vi "Drive Teleop Handler.vi"(10 "Call Context":T1=enum."Stop") -> ()   [LabVIEW 2027]
uses:
  Drive/Implementation/Driving Mode.ctl
  <vilib>/Rock Robotics/WPI/Joystick/XBox Buttons Indexer.ctl
  swerve-template/Type Definitions/Data/Robot Velocities.ctl
  fdc21bd4-9215-41b8-8367-bf19dde4ba27.vi
  <vilib>/Rock Robotics/Network Tables/NT Read Number.vi
  Framework/Robot Global Data.vi
  <vilib>/Rock Robotics/WPI/DriverStation/WPI_DriverStationDerivedRobotMode.ctl
  20f039dc-a6f5-4e97-88ba-31848a91c715.vi
  ce51abe2-3967-49ec-91df-d4b8ef358bb3.vi
  <vilib>/Rock Robotics/Network Tables/NT Read Boolean.vi
  2558f998-dd4e-4154-8f44-6f70b21d0474.vi
  <vilib>/Rock Robotics/Network Tables/NT Write Boolean.vi
  <vilib>/MRC/MrcLib.lvlib
panel:
  in  "Max ToF Data":cluster{"ToF":dbl, "Dist":dbl}={"ToF"=1.2, "Dist"=10.52}
  in  "Min ToF Data":cluster{"ToF":dbl, "Dist":dbl}={"ToF"=1.0, "Dist"=6.0}
  in  "Time in Flight":dbl=1.1
  in  "Max Translation Align":dbl=4.0
  in  "Deadband Info":T2={"Deadband"=0.05, "Deadband High"=1.0, "Deadband Low"=0.05}
  in  "Max Velocities":T3={"X Velocity"=15.0, "Y Velocity"=15.0, "Rotational \nVelocity"=270.0}
  in  "Sinusoidal Terms":cluster{"Max Velocity":dbl, "Frequency":dbl}
  in  "Teleop Mode":T4(ring)
  in  "Joystick Inputs":T5(array[cluster])
  in  "Send Inputs":bool
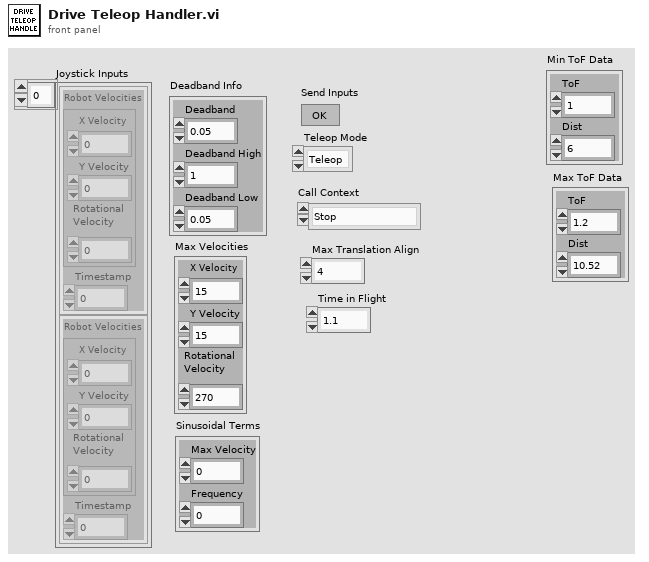
[diagram p1: front panel]
types:
  T1 = typedef "WPI_DriverStationDerivedRobotMode.ctl" = enum16{"Init", "Execute", "Stop"}
  T2 = cluster{"Deadband":dbl, "Deadband High":dbl, "Deadband Low":dbl}
  T3 = typedef "Robot Velocities.ctl" = cluster{"X Velocity":dbl, "Y Velocity":dbl, "Rotational \nVelocity":dbl}
  T4 = enum16{"Teleop", "Simulated Teleop", "Sine Velocity Profiles", "Circle Simulator"}
  T5 = cluster{"Robot Velocities":T3, "Timestamp":dbl}[]
  T6 = typedef "XBox Buttons Indexer.ctl" = enum16{"A", "B", "X", "Y", "Left Bumper", "Right Bumper", "Back", "Start", "Left Joystick", "Right Joystick"}
  T7 = typedef "Driving Mode.ctl" = enum16{"Robot Centric", "Field Centric"}
  T8 = typedef "WPI_JoystickDevRef.ctl" = cluster{"Device":T9}
  T9 = typedef "WPI_JoystickDeviceEnum.ctl" = enum16{"USB 0", "USB 1", "USB 2", "USB 3", "USB 4", "USB 5"}
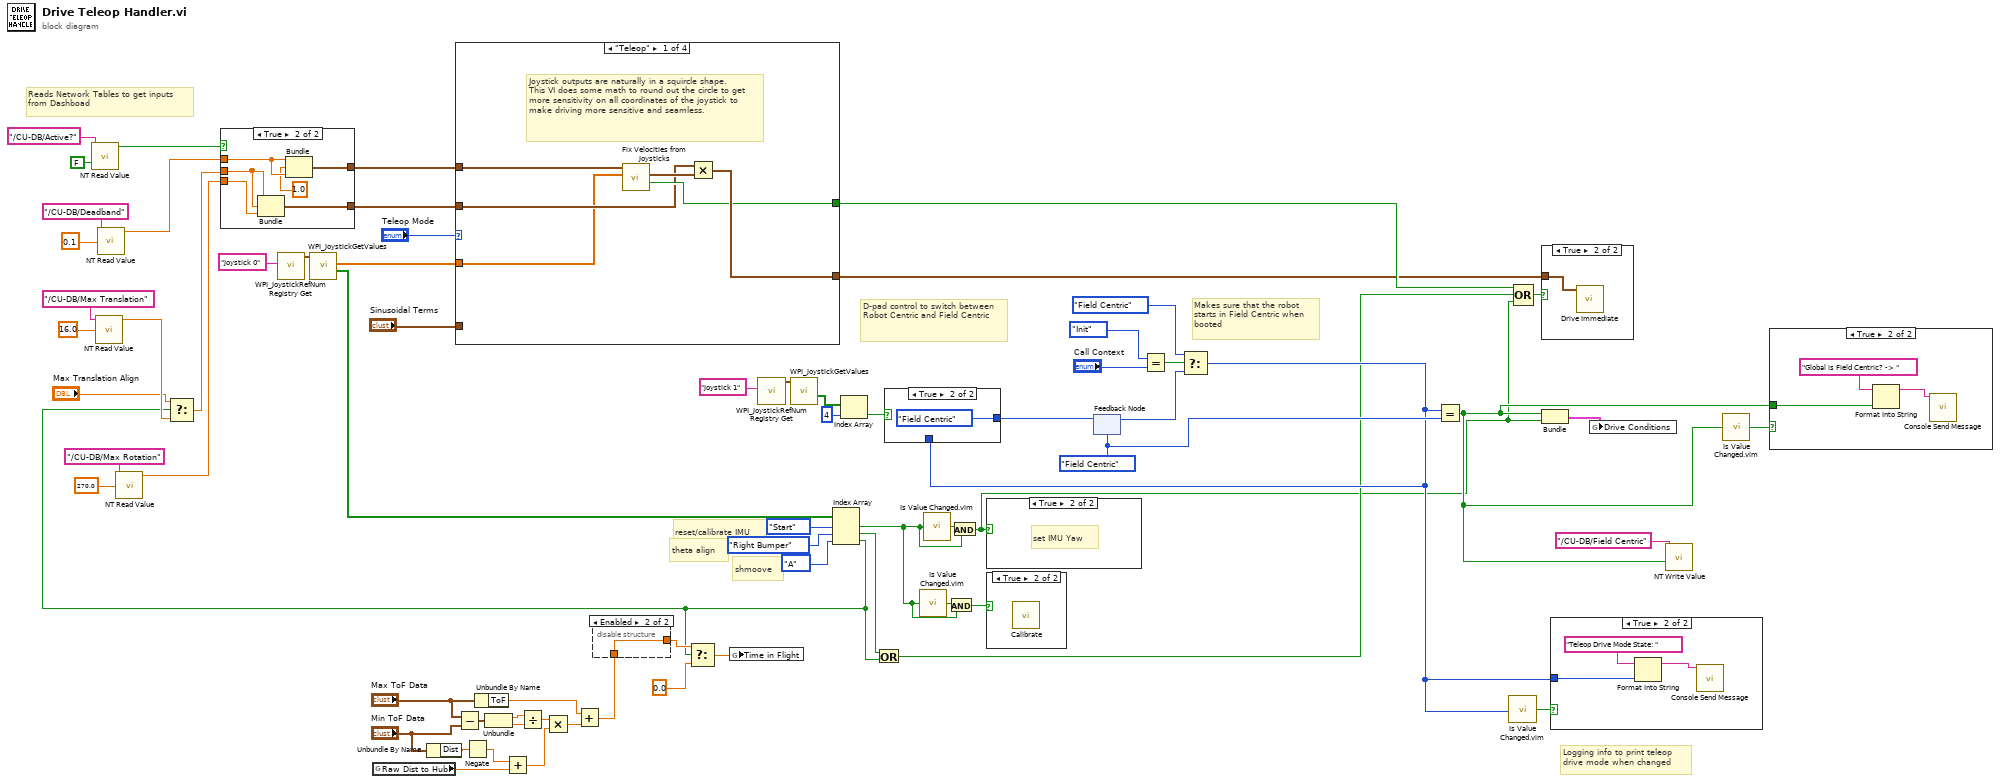
[diagram p0: block diagram]
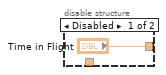
[diagram p2: hidden frame]
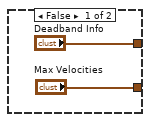
[diagram p8: hidden frame]
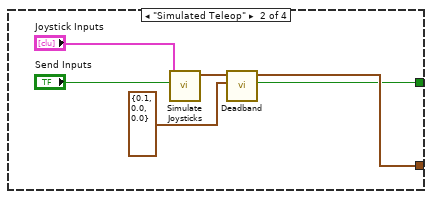
[diagram p9: hidden frame]
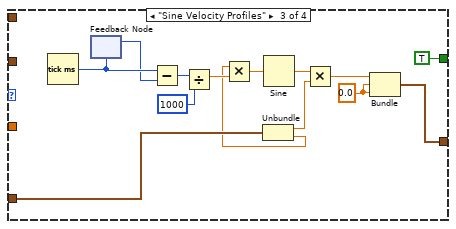
[diagram p10: hidden frame]
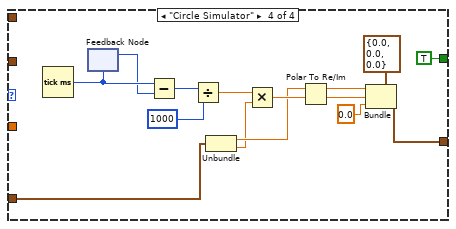
[diagram p11: hidden frame]
diagram:
  w41 = Driving_Mode."Field Centric"
  # "shmoove"
  # "theta align"
  # "reset/calibrate IMU"
  # "Reads Network Tables to get inputs from Dashboad"
  # "Logging info to print teleop drive mode when changed"
  # "Makes sure that the robot starts in Field Centric when booted"
  # "D-pad control to switch between Robot Centric and Field Centric"
  n1 = call-poly <vilib>:"NT Read Value.vi"("default value"=FALSE ("Default Value"), "name"="/CU-DB/Active?" ("Name")) -> ("value"=w53:bool)  [unwired: 7 in, 2 out]
  n2 = call-poly <vilib>:"NT Read Value.vi"("default value"=16.0 ("Default Value"), "name"="/CU-DB/Max Translation" ("Name")) -> ("value"=w28:dbl)  [unwired: 7 in, 2 out]
  n3 = call-poly <vilib>:"NT Read Value.vi"("default value"=0.1 ("Default Value"), "name"="/CU-DB/Deadband" ("Name")) -> ("value"=w52:dbl)  [unwired: 7 in, 2 out]
  n4 = call-poly <vilib>:"NT Read Value.vi"("default value"=270.0 ("Default Value"), "name"="/CU-DB/Max Rotation" ("Name")) -> ("value"=w50:dbl)  [unwired: 7 in, 2 out]
  n5 = call <vilib>:"WPI_JoystickRefNum Registry Get.vi"("refnum name"="Joystick 0") -> ("JoystickDevRef"=w69:T8)  [unwired: 1 in, 9 out]
  n6 = call <vilib>:"WPI_JoystickGetValues.vi"("JoystickDevRef"=w69) -> ("Buttons"=w66:bool[], "Axes"=w68:dbl[])  [unwired: 6 in, 3 out]
  n7 = global read "Robot Global Data.vi" "Raw Dist to Hub"() -> (w5:dbl)
  n8 = Unbundle By Name("Min ToF Data") -> ("Dist"=w6:dbl)
  n9 = Subtract(x="Max ToF Data", y="Min ToF Data") -> (x-y=w14:cluster{"ToF":dbl, "Dist":dbl})
  n10 = Negate(x=w6) -> (-x=w4:dbl)
  n11 = Unbundle By Name("Max ToF Data") -> ("ToF"=w8:dbl)
  n12 = Unbundle(w14) -> ("ToF"=w13:dbl, "Dist"=w12:dbl)
  n13 = Add(x=w4, y=w5) -> (x+y=w3:dbl)
  n14 = Divide(x=w13, y=w12) -> (x/y=w11:dbl)
  n15 = Multiply(x=w11, y=w3) -> (x*y=w10:dbl)
  n16 = Add(x=w8, y=w10) -> (x+y=w2:dbl)
  n17 = disable-structure shown="Enabled" {
    disable-tunnel: ["Time in Flight" w72] -> w17
    disable-tunnel: w2 -> [_ w72]
    frame Disabled {
    }
    frame Enabled {
    }
  }
  n18 = call <vilib>:"WPI_JoystickRefNum Registry Get.vi"("refnum name"="Joystick 1") -> ("JoystickDevRef"=w25:T8)  [unwired: 1 in, 9 out]
  n19 = call <vilib>:"WPI_JoystickGetValues.vi"("JoystickDevRef"=w25) -> ("Buttons"=w23:bool[])  [unwired: 6 in, 4 out]
  n20 = Index Array(array=w66, index #1=XBox_Buttons_Indexer."Start" ("XBox Buttons"), index #2=XBox_Buttons_Indexer."Right Bumper" ("XBox Buttons"), index #3=XBox_Buttons_Indexer."A" ("XBox Buttons")) -> (element #1=w33:bool, element #2=w20:bool, element #3=w16:bool)
  n21 = Select(t="Max Translation Align", s=w16, f=w28) -> (s? t:f=w29:dbl)
  n22 = case shown="True" w53 {
    tunnel: w52 -> [_ w80]
    tunnel: ["Deadband Info" w78] -> w51
    tunnel: w29 -> [_ w77]
    tunnel: w50 -> [_ w76]
    tunnel: ["Max Velocities" w75] -> w49
    frame False {
    }
    frame True {
      n23 = Bundle("value"=w77, "value"=w77, "value"=w76) -> (w75:cluster{"value":dbl, "value":dbl, "value":dbl})  [unwired: 1 in]
      n24 = Bundle("value"=w80, "value"=1.0, "value"=w80) -> (w78:cluster{"value":dbl, "value":dbl, "value":dbl})  [unwired: 1 in]
    }
  }
  n25 = case shown="\"Teleop\"" "Teleop Mode" {
    tunnel: w68 -> [w81 _ _ _]
    tunnel: [w86 w92 w97 w119] -> w31
    tunnel: "Sinusoidal Terms" -> [_ _ w96 w109]
    tunnel: w51 -> [w85 _ _ _]
    tunnel: w49 -> [w82 _ _ _]
    tunnel: [w83 w87 TRUE ("Sending Input?") TRUE ("Sending Input?")] -> w47
    frame "Teleop" {
      # "Joystick outputs are naturally in a squircle shape.\nThis VI does some math to round out the circle to get more sensitivity on all coordinates of the joystick to make driving more sensitive and seamless."
      n26 = call "Fix Velocities from Joysticks.vi"("Axes"=w81, "Deadband"=w85) -> ("Sending Input?"=w83:bool, "Adjusted Robot Velocities"=w84:T3)  [unwired: 8 in]
      n27 = Multiply(x=w82, y=w84) -> (x*y=w86:T3)
    }
    frame "Simulated Teleop" {
      n28 = call "Simulate Joysticks.vi"("Send Inputs"="Send Inputs", "Joystick Inputs"="Joystick Inputs") -> ("Joystick Inputs"=w89:T3)  [unwired: 9 in]
      n29 = call "Deadband.vi"("Deadband Info"=T2 {"Deadband"=0.1, "Deadband High"=0.0, "Deadband Low"=0.0}, "Robot Velocities"=w89) -> ("Sending Input?"=w87:bool, "Adjusted Robot Velocities"=w92:T3)  [unwired: 8 in]
    }
    frame "Sine Velocity Profiles" {
      w105 = 0.0
      n30 = Tick Count (ms)() -> (millisecond timer value=w99:u32)
      n31 = feedback #1(w99) -> (w98:u32)
      n32 = feedback-in #1(w98) -> ()
      n33 = Subtract(x=w99, y=w98) -> (x-y=w103:u32)
      n34 = Divide(x=w103, y=u32 1000) -> (x/y=w101:dbl)
      n35 = Unbundle(w96) -> ("Max Velocity"=w94:dbl, "Frequency"=w95:dbl)
      n36 = Multiply(x=w95, y=w101) -> (x*y=w100:dbl)
      n37 = Sine(x=w100) -> (sin(x)=w104:dbl)
      n38 = Multiply(x=w104, y=w94) -> (x*y=w106:dbl)
      n39 = Bundle(w106, w105, w105) -> (w97:cluster{dbl, dbl, dbl})  [unwired: 1 in]
    }
    frame "Circle Simulator" {
      n40 = Tick Count (ms)() -> (millisecond timer value=w115:u32)
      n41 = feedback #2(w115) -> (w114:u32)
      n42 = feedback-in #2(w114) -> ()
      n43 = Subtract(x=w115, y=w114) -> (x-y=w117:u32)
      n44 = Divide(x=w117, y=u32 1000) -> (x/y=w111:dbl)
      n45 = Unbundle(w109) -> ("Max Velocity"=w112:dbl, "Frequency"=w110:dbl)
      n46 = Multiply(x=w111, y=w110) -> (x*y=w113:dbl)
      n47 = Polar To Re/Im(2:w113, 3:w112) -> (0:w107:dbl, 1:w108:dbl)
      n48 = Bundle(cluster=T3 {"X Velocity"=0.0, "Y Velocity"=0.0, "Rotational \nVelocity"=0.0} ("Robot Velocities (ft/s and deg/s)"), "X Velocity"=w108, "Y Velocity"=w107, "Rotational \nVelocity"=0.0 ("Rotational \nVelocity")) -> (w119:T3)
    }
  }
  n49 = Select(t=w17, s=w16, f=0.0) -> (s? t:f=w18:dbl)
  n50 = global write "Robot Global Data.vi" "Time in Flight"(w18) -> ()
  n51 = Index Array(array=w23, index=4) -> (element=w22:bool)
  n52 = Or(x=w20, y=w16) -> (x .or. y?=w19:bool)
  n53 = call "Is Value Changed.vim"("value"=w33) -> ("changed or first call?"=w36:bool)
  n54 = call "Is Value Changed.vim"("value"=w33) -> ("changed or first call?"=w64:bool)
  n55 = And(x=w36, y=w33) -> (x .and. y?=w35:bool)
  n56 = And(x=w64, y=w33) -> (x .and. y?=w1:bool)
  n57 = case shown="True" w1 {
    selector: w1 -> [_ w122]
    frame False {
    }
    frame True {
      # "set IMU Yaw"
    }
  }
  n58 = case shown="True" w35 {
    frame False {
    }
    frame True {
      n59 = call "Calibrate.vi"() -> ()  [unwired: 11 in, 1 out]
    }
  }
  n60 = feedback #3(w41) -> (w40:T7)
  n61 = Equal?(x=WPI_DriverStationDerivedRobotMode."Init" ("y"), y="Call Context") -> (x = y?=w43:bool)
  n62 = Select(t=Driving_Mode."Field Centric" ("x"), s=w43, f=w40) -> (s? t:f=w38:T7)
  n63 = case shown="True" w22 {
    tunnel: [w123 Driving_Mode."Field Centric"] -> w67
    tunnel: w38 -> [w123 _]
    frame False {
    }
    frame True {
    }
  }
  n64 = feedback-in #3(w67) -> ()
  n65 = Equal?(x=w38, y=w41) -> (x = y?=w30:bool)
  n66 = call "Is Value Changed.vim"("value"=w38) -> ("changed or first call?"=w37:bool)
  n67 = Compound Arithmetic op=OR(w47, w19, w1) -> (w48:bool)
  n68 = case shown="True" w48 {
    tunnel: w31 -> [_ w125]
    frame False {
    }
    frame True {
      n69 = call "Drive Immediate.vi"("Robot Velocities"=w125) -> ()  [unwired: 10 in, 1 out]
    }
  }
  n70 = Bundle(w30, w1) -> (w34:cluster{bool, bool})  [unwired: 1 in]
  n71 = case shown="True" w37 {
    tunnel: w38 -> [_ w127]
    frame False {
    }
    frame True {
      n72 = Format Into String(initial string="Teleop Drive Mode State: ", w127) -> (resulting string=w126:string)  [unwired: 2 in, 1 out]
      n73 = call <vilib>:"Console Send Message.vi"("Message"=w126) -> ()  [unwired: 14 in, 1 out]
    }
  }
  n74 = global write "Robot Global Data.vi" "Drive Conditions"(w34) -> ()
  n75 = call-poly <vilib>:"NT Write Value.vi"("value"=w30, "name"="/CU-DB/Field Centric") -> ()  [unwired: 9 in, 1 out]
  n76 = call "Is Value Changed.vim"("value"=w30) -> ("changed or first call?"=w39:bool)
  n77 = case shown="True" w39 {
    tunnel: w30 -> [_ w131]
    frame False {
    }
    frame True {
      n78 = Format Into String(initial string="Global is Field Centric? -> ", w131) -> (resulting string=w129:string)  [unwired: 2 in, 1 out]
      n79 = call <vilib>:"Console Send Message.vi"("Message"=w129) -> ()  [unwired: 14 in, 1 out]
    }
  }
